vi "PicoScope2000GetValues.vi"(5 "enabled array":i16[](array[numeric]), 7 "Buffer and Transfer Settings":T1={"startIndex"=0, "Samples"=2000, "Down Sample Ratio"=1, "Down-Sample Mode"=0} {"Down-Sample Mode" items=["RAW none"=2147483648, "None"=0, "Aggregate"=1, "Decimate"=2, "Average"=4]; "Down Sample Ratio" step=1; "Samples" format="%_6p"}, 8 "error in (no error)":errorcluster, 10 "Data Pointers In":T2, 11 "handle in":i16) -> (0 "error out":errorcluster, 3 "handle out":i16, 4 "overflow":i16 format="%010b", 6 "noOfSamples":u64)   [LabVIEW 2010]
doc: "Calls ps5000aGetValuesOverlapped"
uses:
  ps2000.dll
  shared/PicoBuffers.ctl
  shared/Buffer and Transfer Settings.ctl
panel:
  out "numSamples":i32
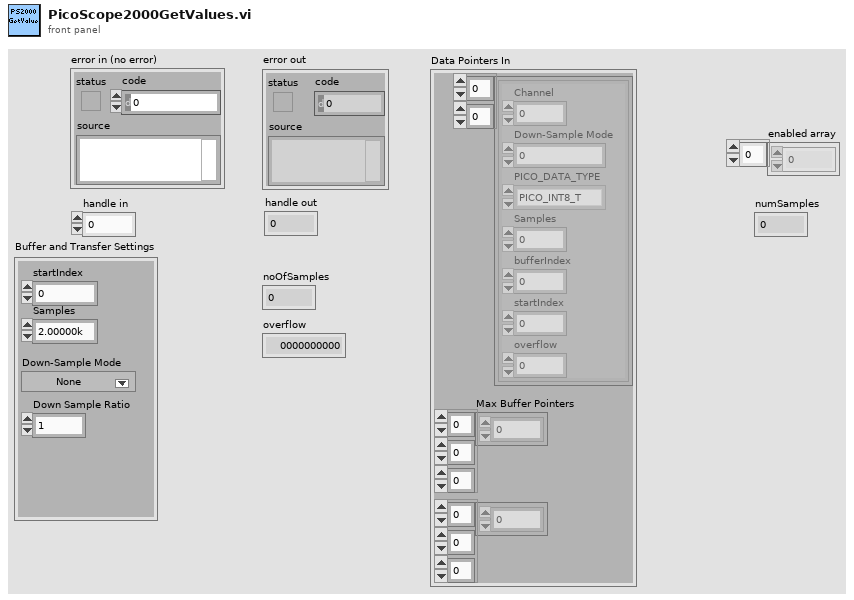
[diagram p1: front panel]
types:
  T1 = typedef "Buffer and Transfer Settings.ctl" = cluster{"startIndex":u64, "Samples":u64, "Down Sample Ratio":u64, "Down-Sample Mode":u32}
  T2 = typedef "PicoBuffers.ctl" = cluster{"Max Buffer Pointers":u64[][][], "Min Buffer Pointers":u64[][][], "StreamingDataInfo":cluster{"Channel":u32, "Down-Sample Mode":u32, "PICO_DATA_TYPE":enum32{"PICO_INT8_T", "PICO_INT16_T", "PICO_INT32_T", "PICO_UINT32_T", "PICO_INT64_T", ""}, "Samples":i32, "bufferIndex":u64, "startIndex":i32, "overflow":i16}[][]}
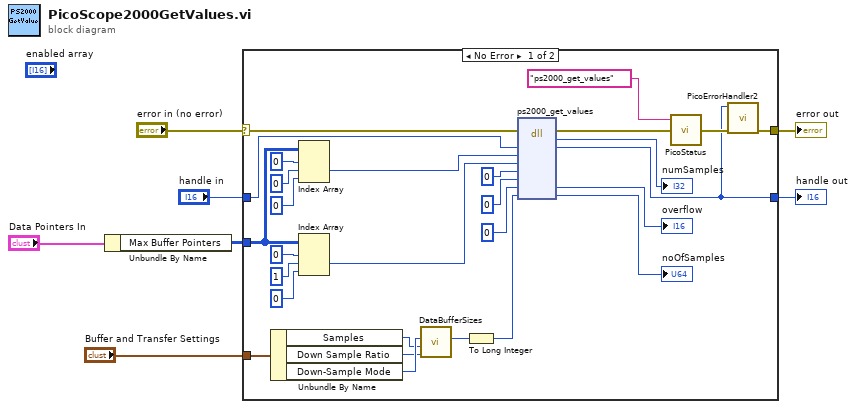
[diagram p0: block diagram]
diagram:
  n1 = Unbundle By Name("Data Pointers In") -> ("Max Buffer Pointers"=w4:u64[][][])
  n2 = case shown="No Error" "error in (no error)" {
    selector: "error in (no error)" -> [w31 w36]
    tunnel: "handle in" -> [w30 w37]
    tunnel: [w29 w37] -> w2
    tunnel: [w33 w36] -> w3
    tunnel: w4 -> [w14 _]
    tunnel: "Buffer and Transfer Settings" -> [w9 _]
    frame No Error {
      n3 = Unbundle By Name(w9) -> ("Samples"=w11:u64, "Down Sample Ratio"=w10:u64, "Down-Sample Mode"=w12:u32)
      n4 = Index Array(array=w14, index (dim 0)=0 ("index (page)"), index (dim 1)=0 ("disabled index (row)"), index (dim 2)=0 ("disabled index (col)")) -> (element=w15:u64)
      n5 = Index Array(array=w14, index (dim 0)=0 ("index (page)"), index (dim 1)=1 ("disabled index (row)"), index (dim 2)=0 ("disabled index (col)")) -> (element=w19:u64)
      n6 = call "DataBufferSizes.vi"("Down Sample Ratio"=w10, "Number of Samples"=w11, "Down-Sample Mode"=w12) -> ("Max Buffer Size"=w8:i32)  [unwired: 7 in, 1 out]
      n7 = To Long Integer(number=w8) -> (32bit integer=w13:i32)
      n8 = dll-call lib="PS2000.dll" fn="ps2000_get_values"(error in=w31, "handle"=w30, "bufferA"=w15, "bufferB"=w19, "bufferC"=u64 0, "bufferD"=u64 0, "overflow"=i16 0, "numValues"=w13) -> (error out=w32:errorcluster, "numSamples"=→"numSamples":i32, "handle"=w29:i16, "overflow"=→"overflow":i16, "numValues"=→"noOfSamples":i32)  [unwired: 6 in, 1 out]
      n9 = call "PicoStatus.vi"("error in"=w32, "source"="ps2000_get_values") -> ("error out"=w35:errorcluster)  [unwired: 1 in]
      n10 = call "PicoErrorHandler2.vi"("error in (no error)"=w35, "handle In"=w29) -> ("error out"=w33:errorcluster)  [unwired: 9 in]
    }
    frame Error {
    }
  }
  "error out" <- w3
  "handle out" <- w2
